vi "CARRIERSIGNAL...vi"() -> (11 "Waveform Graph":dbl[](graph))   [LabVIEW 2023]
panel:
  in  "Numeric":i32
  in  "sampling frequency":dbl
  in  "number of samples":dbl
  in  "carrier frequency":dbl
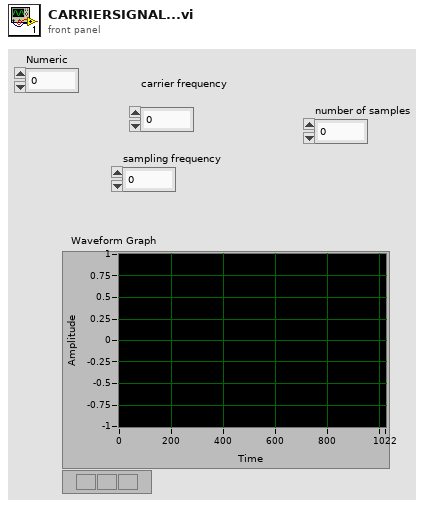
[diagram p1: front panel]
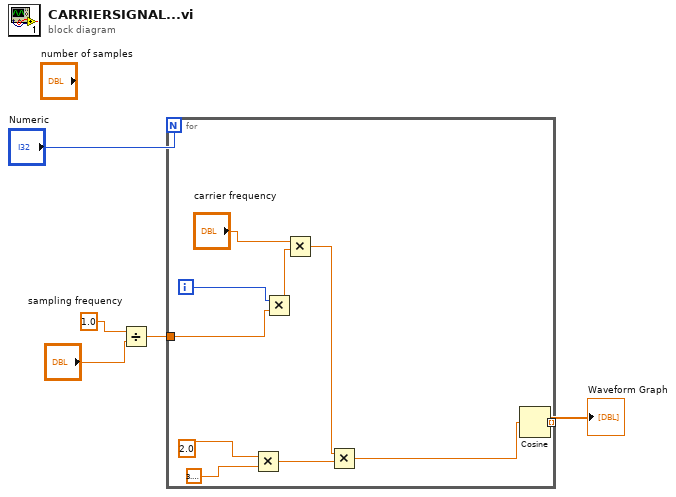
[diagram p0: block diagram]
diagram:
  n1 = Divide(x=1.0, y="sampling frequency") -> (x/y=w2:dbl)
  n2 = for {
    N: "Numeric" -> [_]
    tunnel: [w13] -> w5 mode=indexing
    tunnel: w2 -> [w6]
    i -> [w12]
    n3 = Multiply(x=2.0 ("x*y"), y=3.141592653589793) -> (x*y=w11:dbl)
    n4 = Multiply(x=w12, y=w6) -> (x*y=w10:dbl)
    n5 = Multiply(x="carrier frequency", y=w10) -> (x*y=w9:dbl)
    n6 = Multiply(x=w9, y=w11) -> (x*y=w8:dbl)
    n7 = Cosine(x=w8) -> (cos(x)=w13:dbl)
  }
  "Waveform Graph" <- w5
